vi "Register Events.vi"(8 "error in (no error)":errorcluster, 11 "PluginGUI in":refnum<class "PluginGUI.lvclass">) -> (0 "error out":errorcluster, 3 "PluginGUI out":refnum<class "PluginGUI.lvclass">)   [LabVIEW 2020, in "VolatusGUI.lvlib" / "PluginGUI.lvclass"]
uses:
  PluginGUI.lvclass
  Control Event.ctl
  PluginGUI.lvclass/PluginGUI.ctl
  <vilib>/Utility/miscctls.llb/LVMapReplaceAction.ctl
  VolatusGUI.lvlib
  GUI Element/GUI Element.lvclass
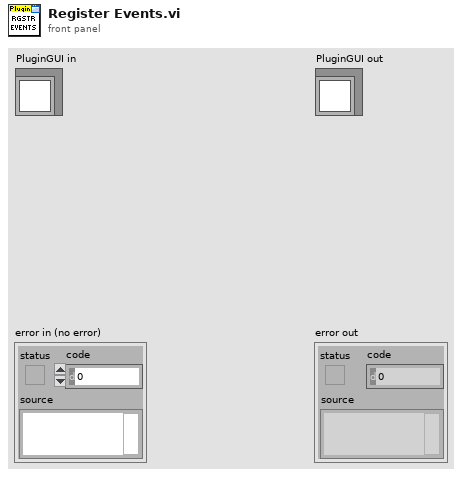
[diagram p1: front panel]
types:
  T1 = typedef "VolatusGUI.lvlib/Control Event.ctl" = enum16{"Value Change", "Shortcut Menu", "Mouse Down"}
  T2 = typedef "LVMapReplaceAction.ctl" = enum32{"Modify Entry only if found", "Add or Modify Entry", "Delete Entry"}
  T3 = typedef "VolatusGUI.lvlib/Event Registration.ctl" = cluster{"CtlRef":refnum<vi>, "Event":T1}
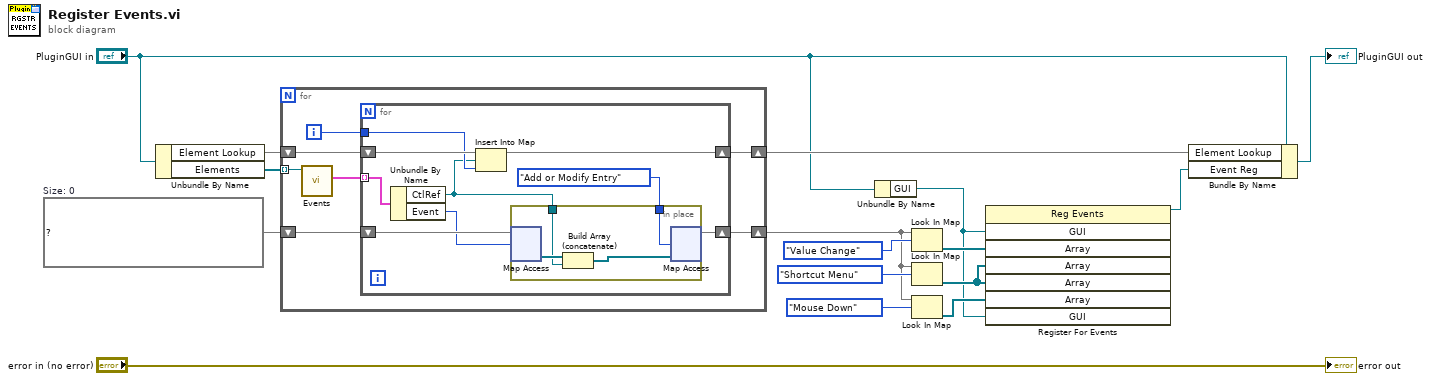
[diagram p0: block diagram]
diagram:
  w14 = map{T1, refnum<vi>[]} {}  # Size: 0
  n1 = Unbundle By Name("PluginGUI in") -> ("Element Lookup"=w15:map{refnum<vi>, i32}, "Elements"=w16:refnum<class "GUI Element.lvclass">[])
  n2 = for {
    tunnel: w16 -> [w23] mode=indexing
    shift-right: [w18] -> w8
    shift-left: w15 -> [w22]
    shift-right: [w17] -> w6
    shift-left: w14 -> [w20]
    i -> [w19]
    n3 = call "Events.vi"("GUI Element in"=w23) -> ("Events"=w21:T3[])  [unwired: 10 in]
    n4 = for {
      shift-right: [w29] -> w18
      shift-left: w22 -> [w31]
      tunnel: w21 -> [w32] mode=indexing
      shift-right: [w24] -> w17
      shift-left: w20 -> [w28]
      tunnel: w19 -> [w30]
      n5 = Unbundle By Name(w32) -> ("CtlRef"=w26:refnum<vi>, "Event"=w27:T1)
      n6 = Insert Into Map(map in=w31, key=w26, value=w30) -> (map out=w29:map{refnum<vi>, i32})  [unwired: 2 out]
      n7 = in-place {
        in-place-border: w26 -> [w35]
        in-place-border: LVMapReplaceAction."Add or Modify Entry" ("action") -> [w33]
        n8 = in-place-map #1(w28, w27) -> (w36:refnum<vi>[])  [unwired: 1 in, 1 out]
        n9 = Build Array (concatenate)(w36, w35) -> (w34:refnum<vi>[])
        n10 = in-place-map #1(w34, w33) -> (w24:map{T1, refnum<vi>[]})  [unwired: 2 out]
      }
    }
  }
  n11 = Unbundle By Name("PluginGUI in") -> ("GUI"=w2:refnum<vi>)
  n12 = Look In Map(map=w6, key=Control_Event."Value Change") -> (value=w11:refnum<vi>[])  [unwired: 1 in, 1 out]
  n13 = Look In Map(map=w6, key=Control_Event."Shortcut Menu") -> (value=w10:refnum<vi>[])  [unwired: 1 in, 1 out]
  n14 = Look In Map(map=w6, key=Control_Event."Mouse Down") -> (value=w4:refnum<vi>[])  [unwired: 1 in, 1 out]
  n15 = register-events(w2, w11, w10, w10, w4, w2) -> (reference out=w1:refnum<event-registration>)  [unwired: 2 in, 1 out]
  n16 = Bundle By Name(cluster="PluginGUI in", "Element Lookup"=w8, "Event Reg"=w1) -> (→"PluginGUI out":refnum<class "PluginGUI.lvclass">)
  "error out" <- "error in (no error)"
